vi "VIH Utility - STR - String to 1D Str Array (w delimiter pattern).vi"(6 "Delimiter pattern ([\\s\\t]+)":string="[\\s\\t]+", 7 "String":string) -> (3 "Array out":string[](array[string]))   [LabVIEW 2014]
doc: "::: VI Helpeks :::\nCopyright (c) 2000-2026 Konstantin Shifershteyn. All rights reserved."
panel:
  # "VI Helpeks\nCopyright (c) 2012-2026 Konstantin Shifershteyn"
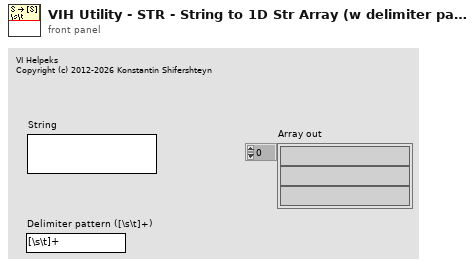
[diagram p1: front panel]
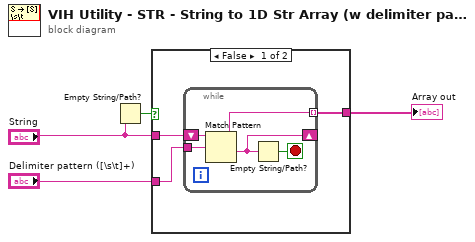
[diagram p0: block diagram]
diagram:
  n1 = Empty String/Path?(string/path="String") -> (empty?=w1:bool)
  n2 = case shown="False" w1 {
    tunnel: "String" -> [w7 _]
    tunnel: [w6 _] -> w4
    tunnel: "Delimiter pattern ([\\s\\t]+)" -> [w5 _]
    frame False {
      n3 = while {
        shift-right: [w10] -> _
        shift-left: w7 -> [w12]
        tunnel: [w11] -> w6 mode=indexing
        tunnel: w5 -> [w8]
        stop <- w9 stop-if-true
        n4 = Match Pattern(string=w12, regular expression=w8) -> (before substring=w11:string, after substring=w10:string)  [unwired: 3 out]
        n5 = Empty String/Path?(string/path=w10) -> (empty?=w9:bool)
      }
    }
    frame True {
    }
  }
  "Array out" <- w4
